vi "PicoScopeospaAdvancedTriggerPWQ.vi"(0 "handle in":i16=16384, 1 "Pulse Width Qualifier Settings":T3 {"Pulse Width Type" items=["None", "Less Than", "Greater Than", "In Range", "Out of Range"]}, 2 "Pulse Width Qualifier Trigger Properties":T1={"Channel A Trigger Properties"={"Threshold Mode"=0, "Available"=TRUE, "Direction"=2}, "Channel B Trigger Properties"={"Threshold Mode"=0, "Available"=FALSE, "Direction"=2}, "Channel C Trigger Properties"={"Threshold Mode"=0, "Available"=FALSE, "Direction"=2}, "Channel D Trigger Properties"={"Threshold Mode"=0, "Available"=FALSE, "Direction"=2}, "Channel E Trigger Properties"={"Threshold Mode"=0, "Available"=FALSE, "Direction"=2}, "Channel F Trigger Properties"={"Threshold Mode"=0, "Available"=FALSE, "Direction"=2}, "Channel G Trigger Properties"={"Threshold Mode"=0, "Available"=FALSE, "Direction"=2}, "Channel H Trigger Properties"={"Threshold Mode"=0, "Available"=FALSE, "Direction"=2}, "Port 0 Trigger Properties"={"Threshold Mode"=0, "Available"=FALSE, "Direction"=2}, "Port 1 Trigger Properties"={"Threshold Mode"=0, "Available"=FALSE, "Direction"=2}} {"Port 1 Trigger Properties"."Direction" items=["Rising"=2, "Falling"=3, "Rising Lower"=7, "Above"=0, "Below"=1, "Rising or Falling"=4, "Falling Lower"=8, "Below Lower"=6, "Above Lower"=5]; "Port 1 Trigger Properties"."Threshold Mode" items=["Level", "Window"]; "Port 0 Trigger Properties"."Direction" items=["Rising"=2, "Falling"=3, "Rising Lower"=7, "Above"=0, "Below"=1, "Rising or Falling"=4, "Falling Lower"=8, "Below Lower"=6, "Above Lower"=5]; "Port 0 Trigger Properties"."Threshold Mode" items=["Level", "Window"]; "Channel H Trigger Properties"."Direction" items=["Rising"=2, "Falling"=3, "Rising Lower"=7, "Above"=0, "Below"=1, "Rising or Falling"=4, "Falling Lower"=8, "Below Lower"=6, "Above Lower"=5]; "Channel H Trigger Properties"."Threshold Mode" items=["Level", "Window"]; "Channel G Trigger Properties"."Direction" items=["Rising"=2, "Falling"=3, "Rising Lower"=7, "Above"=0, "Below"=1, "Rising or Falling"=4, "Falling Lower"=8, "Below Lower"=6, "Above Lower"=5]; "Channel G Trigger Properties"."Threshold Mode" items=["Level", "Window"]; "Channel F Trigger Properties"."Direction" items=["Rising"=2, "Falling"=3, "Rising Lower"=7, "Above"=0, "Below"=1, "Rising or Falling"=4, "Falling Lower"=8, "Below Lower"=6, "Above Lower"=5]; "Channel F Trigger Properties"."Threshold Mode" items=["Level", "Window"]; "Channel E Trigger Properties"."Direction" items=["Rising"=2, "Falling"=3, "Rising Lower"=7, "Above"=0, "Below"=1, "Rising or Falling"=4, "Falling Lower"=8, "Below Lower"=6, "Above Lower"=5]; "Channel E Trigger Properties"."Threshold Mode" items=["Level", "Window"]; "Channel D Trigger Properties"."Direction" items=["Rising"=2, "Falling"=3, "Rising Lower"=7, "Above"=0, "Below"=1, "Rising or Falling"=4, "Falling Lower"=8, "Below Lower"=6, "Above Lower"=5]; "Channel D Trigger Properties"."Threshold Mode" items=["Level", "Window"]; "Channel C Trigger Properties"."Direction" items=["Rising"=2, "Falling"=3, "Rising Lower"=7, "Above"=0, "Below"=1, "Rising or Falling"=4, "Falling Lower"=8, "Below Lower"=6, "Above Lower"=5]; "Channel C Trigger Properties"."Threshold Mode" items=["Level", "Window"]; "Channel B Trigger Properties"."Direction" items=["Rising"=2, "Falling"=3, "Rising Lower"=7, "Above"=0, "Below"=1, "Rising or Falling"=4, "Falling Lower"=8, "Below Lower"=6, "Above Lower"=5]; "Channel B Trigger Properties"."Threshold Mode" items=["Level", "Window"]; "Channel A Trigger Properties"."Direction" items=["Rising"=2, "Falling"=3, "Rising Lower"=7, "Above"=0, "Below"=1, "Rising or Falling"=4, "Falling Lower"=8, "Below Lower"=6, "Above Lower"=5]; "Channel A Trigger Properties"."Threshold Mode" items=["Level", "Window"]}, 11 "error in":errorcluster, 13 "Pulse Width Qualifier Conditions":T2 {"Port 1" items=["Don't Care", "True", "False"]; "Channel H" items=["Don't Care", "True", "False"]; "Channel G" items=["Don't Care", "True", "False"]; "Channel F" items=["Don't Care", "True", "False"]; "Channel E" items=["Don't Care", "True", "False"]; "Aux" items=["Don't Care", "True", "False"]; "Port 0" items=["Don't Care", "True", "False"]; "Channel D" items=["Don't Care", "True", "False"]; "Channel C" items=["Don't Care", "True", "False"]; "Channel B" items=["Don't Care", "True", "False"]; "Channel A" items=["Don't Care", "True", "False"]; "Condition Logic" items=["AND", "OR", "XOR"]}) -> (4 "handle out":i16=16384, 15 "error out":errorcluster)   [LabVIEW 2010]
doc: "This sub VI is an interface for the advanced trigger features of the oscilloscope to support Pulse width qualifier (PWQ)."
uses:
  ps6000a.dll
  psospa.dll
panel:
  in  "PWQ Info Action XOR":bool=TRUE
  in  "PWQ Info Action OR":bool=TRUE
  # "For Condition Logic Suggested settings;\nFor AND, XOR logic-(parallel triggers)\nUse level-type triggers (Level or Inside/outside Window Triggers)\n\nFor OR logic- (single channel)\nUse edge types (e.g. rising, falling, entering window)"
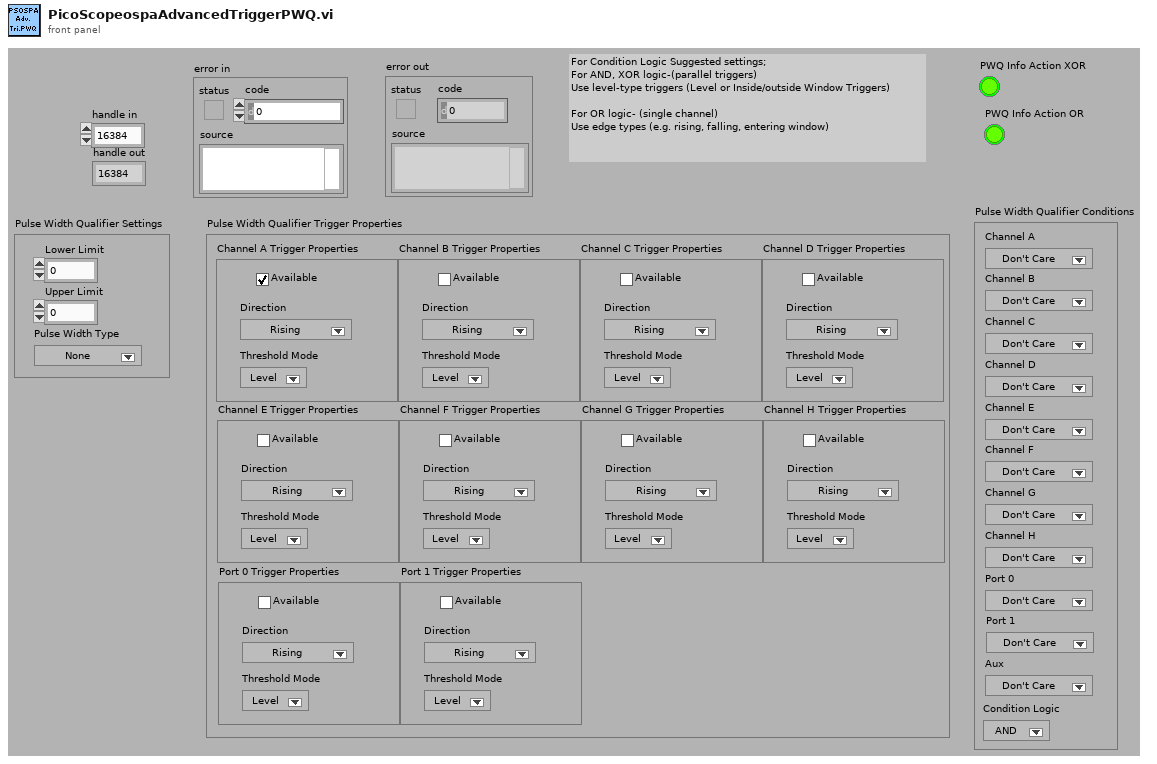
[diagram p1: front panel]
types:
  T1 = cluster{"Channel A Trigger Properties":cluster{"Threshold Mode":i32, "Available":bool, "Direction":u32}, "Channel B Trigger Properties":cluster{"Threshold Mode":i32, "Available":bool, "Direction":u32}, "Channel C Trigger Properties":cluster{"Threshold Mode":i32, "Available":bool, "Direction":u32}, "Channel D Trigger Properties":cluster{"Threshold Mode":i32, "Available":bool, "Direction":u32}, "Channel E Trigger Properties":cluster{"Threshold Mode":i32, "Available":bool, "Direction":u32}, "Channel F Trigger Properties":cluster{"Threshold Mode":i32, "Available":bool, "Direction":u32}, "Channel G Trigger Properties":cluster{"Threshold Mode":i32, "Available":bool, "Direction":u32}, "Channel H Trigger Properties":cluster{"Threshold Mode":i32, "Available":bool, "Direction":u32}, "Port 0 Trigger Properties":cluster{"Threshold Mode":i32, "Available":bool, "Direction":u32}, "Port 1 Trigger Properties":cluster{"Threshold Mode":i32, "Available":bool, "Direction":u32}}
  T2 = cluster{"Channel A":u16, "Channel B":u16, "Channel C":u16, "Channel D":u16, "Channel E":u16, "Channel F":u16, "Channel G":u16, "Channel H":u16, "Port 0":u16, "Port 1":u16, "Aux":u16, "Condition Logic":u16}
  T3 = cluster{"Lower Limit":u32, "Upper Limit":u32, "Pulse Width Type":u32}
  T4 = cluster{"status":bool, "code":u32, "source":string}
  T5 = cluster{"Threshold Mode":i32, "Available":bool, "Direction":u32}[]
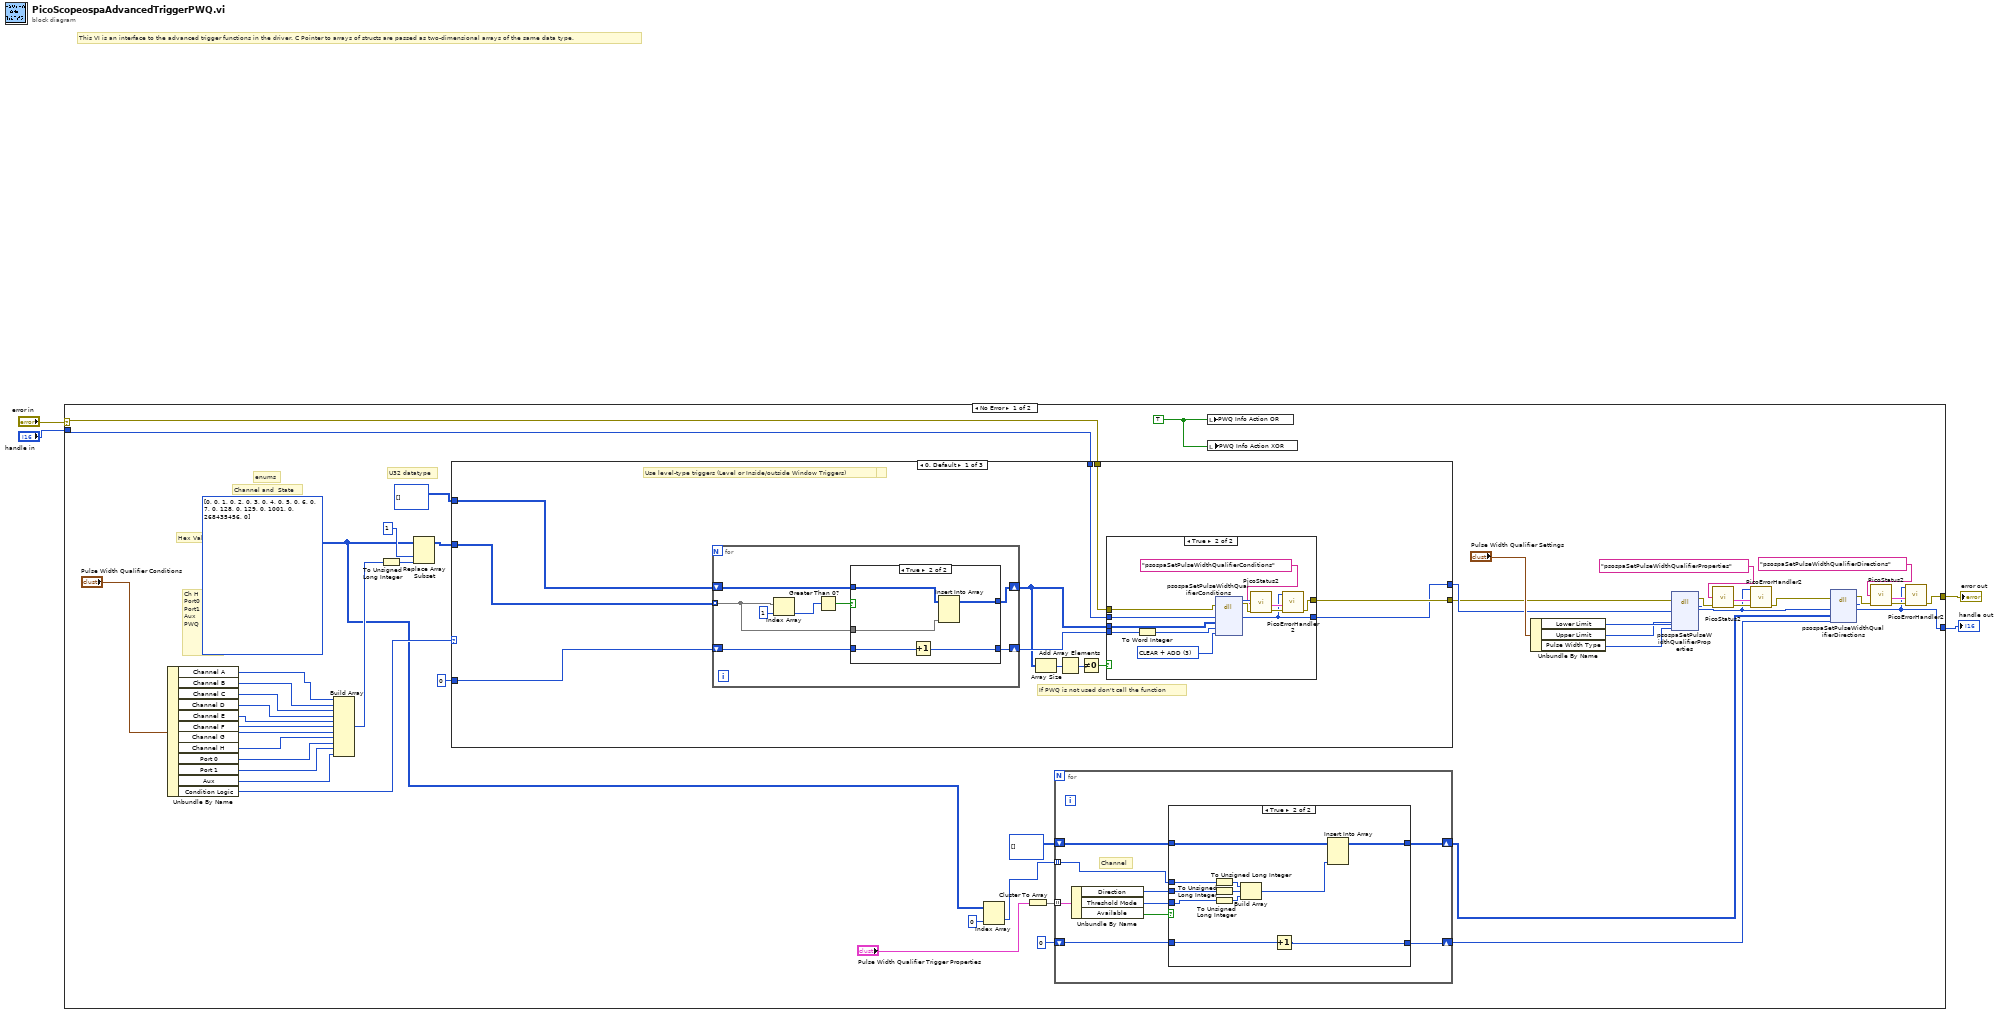
[diagram p0: block diagram]
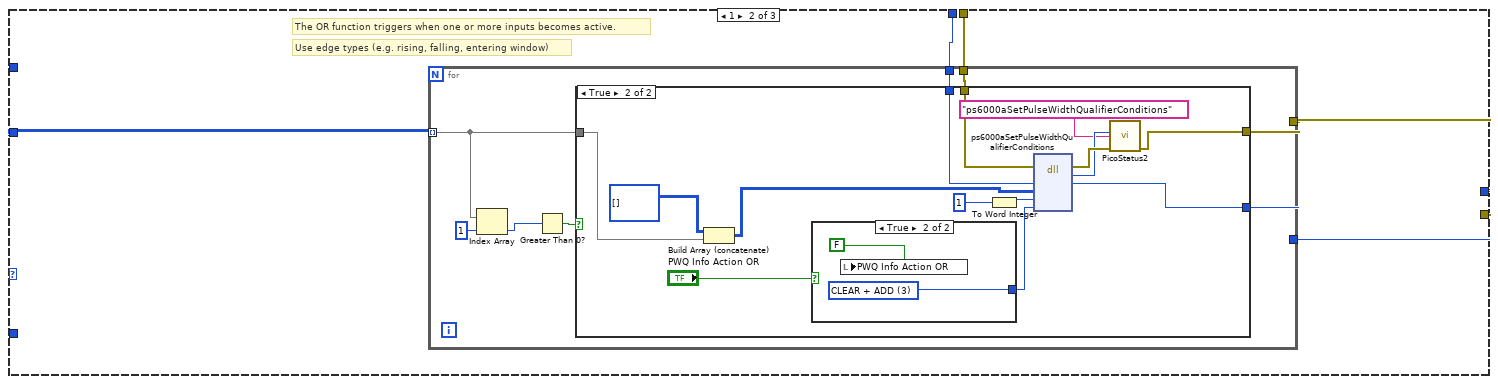
[diagram p5: hidden frame]
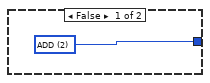
[diagram p7: hidden frame]
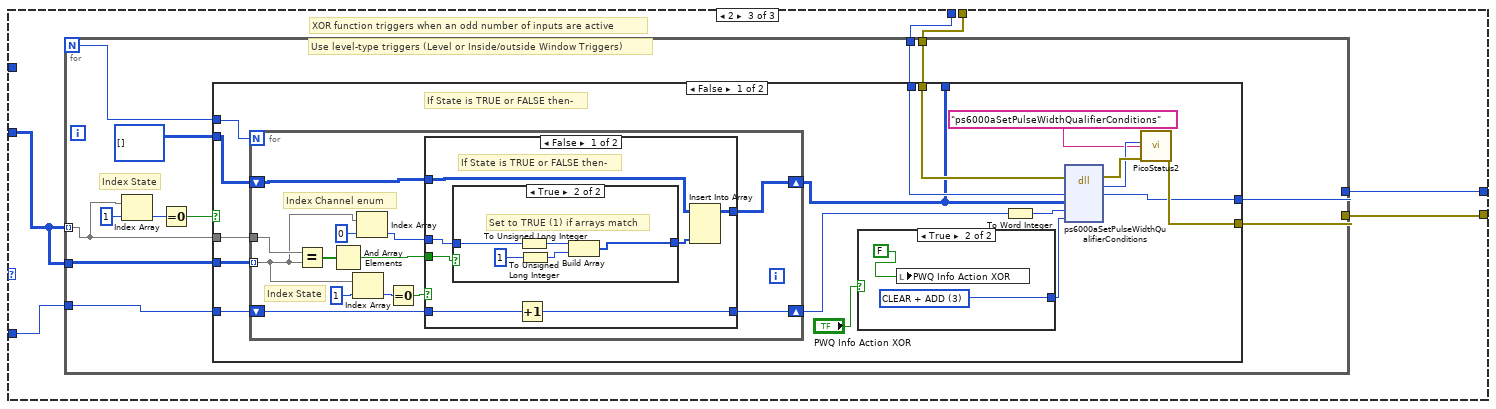
[diagram p8: hidden frame]
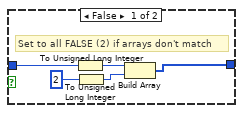
[diagram p9: hidden frame]
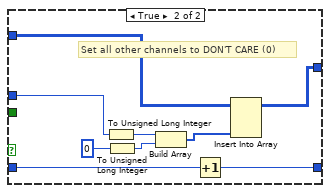
[diagram p10: hidden frame]
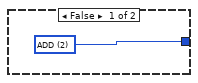
[diagram p11: hidden frame]
diagram:
  # "This VI is an interface to the advanced trigger functions in the driver. C Pointer to arrays of structs are passed as two-dimensional arrays of the same data type."
  n1 = case shown="No Error" "error in" {
    selector: "error in" -> [w14 w232]
    tunnel: "handle in" -> [w13 w233]
    tunnel: [w6 w233] -> w2
    tunnel: [w12 w232] -> w1
    frame No Error {
      w30 = TRUE ("PWQ Info Action XOR")
      w15 = u32[][] [[0, 0], [1, 0], [2, 0], [3, 0], [4, 0], [5, 0], [6, 0], [7, 0], [128, 0], [129, 0], [1001, 0], [268435456, 0]]
      # "U32 datatype"
      # "enums"
      # "Ch H\nPort0\nPort1\nAux\nPWQ"
      # "Channel and  State"
      # "Hex Values"
      n2 = Unbundle By Name("Pulse Width Qualifier Conditions") -> ("Channel A"=w40:u16, "Channel B"=w39:u16, "Channel C"=w38:u16, "Channel D"=w37:u16, "Channel E"=w36:u16, "Channel F"=w35:u16, "Channel G"=w34:u16, "Channel H"=w33:u16, "Port 0"=w32:u16, "Port 1"=w31:u16, "Aux"=w16:u16, "Condition Logic"=w17:u16)
      n3 = Build Array(w40, w39, w38, w37, w36, w35, w34, w33, w32, w31, w16) -> (w54:u16[])
      n4 = To Unsigned Long Integer(number=w54) -> (unsigned 32bit integer=w43:u32[])
      n5 = Replace Array Subset(array=w15, new element=w43, index (col)=1 ("disabled index (col)")) -> (w42:u32[][])  [unwired: 1 in]
      n6 = case shown="0, Default" w17 {
        tunnel: u32[][] [] -> [w89 _ _]
        tunnel: i16 0 -> [w88 _ w152]
        tunnel: w14 -> [w85 w124 w157]
        tunnel: w13 -> [w84 w123 w156]
        tunnel: [w83 w122 w155] -> w44
        tunnel: [w82 w121 w154] -> w45
        tunnel: w42 -> [w86 w120 w153]
        frame 0, Default {
          # "If PWQ is not used don't call the function"
          # "AND function requires both inputs to be active before it will trigger."
          # "Use level-type triggers (Level or Inside/outside Window Triggers)"
          n7 = for {
            shift-right: [w111] -> w87
            shift-left: w88 -> [w110]
            shift-right: [w109] -> w81
            shift-left: w89 -> [w112]
            tunnel: w86 -> [w107] mode=indexing
            n8 = Index Array(array=w107, index=1) -> (element=w106:u32)
            n9 = Greater Than 0?(x=w106) -> (x > 0?=w108:bool)
            n10 = case shown="True" w108 {
              tunnel: w112 -> [w114 w119]
              tunnel: [w114 w118] -> w109
              tunnel: [w113 w117] -> w111
              tunnel: w110 -> [w113 w116]
              tunnel: w107 -> [_ w115]
              frame False {
              }
              frame True {
                n11 = Increment(x=w116) -> (x+1=w117:i16)
                n12 = Insert Into Array(array=w119, new element=w115) -> (w118:u32[][])  [unwired: 2 in]
              }
            }
          }
          n13 = Array Size(array=w81) -> (size(s)=w79:i32[])
          n14 = Add Array Elements(numeric array=w79) -> (sum=w80:i32)
          n15 = Not Equal To 0?(x=w80) -> (x != 0?=w78:bool)
          n16 = case shown="True" w78 {
            tunnel: w87 -> [_ w104]
            tunnel: w85 -> [w91 w100]
            tunnel: w84 -> [w90 w99]
            tunnel: w81 -> [_ w96]
            tunnel: [w91 w95] -> w83
            tunnel: [w90 w92] -> w82
            frame False {
            }
            frame True {
              w98 = u32 3 items=["CLEAR + ADD"=3, "CLEAR"=1, "ADD"=2] ("Condition Action")
              n17 = To Word Integer(number=w104) -> (16bit integer=w97:i16)
              n18 = dll-call lib="psospa.dll" fn="psospaSetPulseWidthQualifierConditions" ("ps3000.dll:_ps3000_open_unit@0")(error in=w100, "handle"=w99, "conditions"=w96, "nConditions"=w97, "action"=w98) -> (error out=w103:errorcluster, "PICO_STATUS"=w102:u32, "handle"=w92:i16)  [unwired: 5 in, 1 out]
              n19 = call "PicoStatus2.vi"("PICO source"="psospaSetPulseWidthQualifierConditions" ("source"), "Error in"=w103, "PICO STATUS"=w102) -> ("error out"=w94:errorcluster, "PICO_STATUS out"=w93:T4)  [unwired: 5 in]
              n20 = call "PicoErrorHandler2.vi"("error in (no error)"=w94, "PICO_STATUS in"=w93, "handle In"=w92) -> ("error out"=w95:errorcluster)  [unwired: 8 in]
            }
          }
        }
        frame 1 {
          # "Use edge types (e.g. rising, falling, entering window)"
          # "The OR function triggers when one or more inputs becomes active."
          n21 = for {
            tunnel: w124 -> [w132]
            tunnel: w123 -> [w131]
            tunnel: [w130] -> w122
            tunnel: [w129] -> w121
            tunnel: w120 -> [w127] mode=indexing
            n22 = Index Array(array=w127, index=1) -> (element=w126:u32)
            n23 = Greater Than 0?(x=w126) -> (x > 0?=w125:bool)
            n24 = case shown="True" w125 {
              tunnel: w132 -> [w133 w144]
              tunnel: w131 -> [w134 w143]
              tunnel: [w133 w141] -> w130
              tunnel: [w134 w140] -> w129
              tunnel: w127 -> [_ w135]
              frame False {
              }
              frame True {
                n25 = Build Array (concatenate)(u32[][] [], w135) -> (w137:u32[][])
                n26 = case shown="True" "PWQ Info Action OR" {
                  tunnel: [w149 w151] -> w142
                  frame False {
                    w149 = u32 2 items=["CLEAR"=1, "ADD"=2, "CLEAR + ADD"=3] ("Condition Action")
                  }
                  frame True {
                    w151 = u32 3 items=["CLEAR"=1, "ADD"=2, "CLEAR + ADD"=3] ("Condition Action")
                    n27 = local write "PWQ Info Action OR"(FALSE ("Boolean")) -> ()
                  }
                }
                n28 = To Word Integer(number=i16 1) -> (16bit integer=w148:i16)
                n29 = dll-call lib="ps6000a.dll" fn="ps6000aSetPulseWidthQualifierConditions" ("ps3000.dll:_ps3000_open_unit@0")(error in=w144, "handle"=w143, "conditions"=w137, "nConditions"=w148, "action"=w142) -> (error out=w147:errorcluster, "PICO_STATUS"=w146:u32, "handle"=w140:i16)  [unwired: 5 in, 1 out]
                n30 = call "PicoStatus2.vi"("PICO source"="ps6000aSetPulseWidthQualifierConditions" ("source"), "Error in"=w147, "PICO STATUS"=w146) -> ("error out"=w141:errorcluster)  [unwired: 5 in, 1 out]
              }
            }
          }
        }
        frame 2 {
          # "Use level-type triggers (Level or Inside/outside Window Triggers)"
          # "XOR function triggers when an odd number of inputs are active"
          n31 = for {
            N -> [w165]
            tunnel: w157 -> [w169]
            tunnel: w156 -> [w168]
            tunnel: [w167] -> w155
            tunnel: [w166] -> w154
            tunnel: w153 -> [w159] mode=indexing
            tunnel: w153 -> [w162]
            tunnel: w152 -> [w163]
            # "Index State"
            n32 = Index Array(array=w159, index=1) -> (element=w160:u32)
            n33 = Equal To 0?(x=w160) -> (x = 0?=w158:bool)
            n34 = case shown="False" w158 {
              tunnel: w169 -> [w186 w229]
              tunnel: w168 -> [w185 w230]
              tunnel: [w184 w229] -> w167
              tunnel: [w183 w230] -> w166
              tunnel: [w181 w231] -> _
              tunnel: w165 -> [w180 _]
              tunnel: u32[][] [] -> [w179 w231]
              tunnel: w163 -> [w178 _]
              tunnel: w162 -> [w177 _]
              tunnel: w159 -> [w176 _]
              frame False {
                # "If State is TRUE or FALSE then-"
                n35 = for {
                  N: w180 -> [_]
                  shift-right: [w198] -> w182
                  shift-left: w178 -> [w199]
                  shift-right: [w187] -> w181
                  shift-left: w179 -> [w188]
                  tunnel: w176 -> [w195]
                  tunnel: w177 -> [w191] mode=indexing
                  # "Index State"
                  # "Index Channel enum"
                  n36 = Equal?(x=w195, y=w191) -> (x = y?=w189:bool[])
                  n37 = And Array Elements(Boolean array=w189) -> (logical AND=w194:bool)
                  n38 = Index Array(array=w191, index=1) -> (element=w192:u32)
                  n39 = Index Array(array=w191, index=0) -> (element=w196:u32)
                  n40 = Equal To 0?(x=w192) -> (x = 0?=w190:bool)
                  n41 = case shown="False" w190 {
                    tunnel: w199 -> [w206 w217]
                    tunnel: [w205 w218] -> w198
                    tunnel: w196 -> [w204 w221]
                    tunnel: w194 -> [w203 _]
                    tunnel: w188 -> [w202 w220]
                    tunnel: [w200 w219] -> w187
                    frame False {
                      # "If State is TRUE or FALSE then-"
                      n42 = case shown="True" w203 {
                        tunnel: [w211 w216] -> w201
                        tunnel: w204 -> [w210 w215]
                        frame False {
                          # "Set to all FALSE (2) if arrays don't match"
                          n43 = To Unsigned Long Integer(number=w210) -> (unsigned 32bit integer=w208:u32)
                          n44 = To Unsigned Long Integer(number=u32 2) -> (unsigned 32bit integer=w209:u32)
                          n45 = Build Array(w208, w209) -> (w211:u32[])
                        }
                        frame True {
                          # "Set to TRUE (1) if arrays match"
                          n46 = To Unsigned Long Integer(number=w215) -> (unsigned 32bit integer=w213:u32)
                          n47 = To Unsigned Long Integer(number=u32 1) -> (unsigned 32bit integer=w214:u32)
                          n48 = Build Array(w213, w214) -> (w216:u32[])
                        }
                      }
                      n49 = Increment(x=w206) -> (x+1=w205:i16)
                      n50 = Insert Into Array(array=w202, new element=w201) -> (w200:u32[][])  [unwired: 2 in]
                    }
                    frame True {
                      # "Set all other channels to DON'T CARE (0)"
                      n51 = To Unsigned Long Integer(number=w221) -> (unsigned 32bit integer=w223:u32)
                      n52 = To Unsigned Long Integer(number=u32 0) -> (unsigned 32bit integer=w224:u32)
                      n53 = Build Array(w223, w224) -> (w225:u32[])
                      n54 = Increment(x=w217) -> (x+1=w218:i16)
                      n55 = Insert Into Array(array=w220, new element=w225) -> (w219:u32[][])  [unwired: 2 in]
                    }
                  }
                }
                n56 = case shown="True" "PWQ Info Action XOR" {
                  tunnel: [w226 w228] -> w170
                  frame False {
                    w226 = u32 2 items=["CLEAR + ADD"=3, "CLEAR"=1, "ADD"=2] ("Condition Action")
                  }
                  frame True {
                    w228 = u32 3 items=["CLEAR + ADD"=3, "CLEAR"=1, "ADD"=2] ("Condition Action")
                    n57 = local write "PWQ Info Action XOR"(FALSE ("Boolean")) -> ()
                  }
                }
                n58 = To Word Integer(number=w182) -> (16bit integer=w175:i16)
                n59 = dll-call lib="ps6000a.dll" fn="ps6000aSetPulseWidthQualifierConditions" ("ps3000.dll:_ps3000_open_unit@0")(error in=w186, "handle"=w185, "conditions"=w181, "nConditions"=w175, "action"=w170) -> (error out=w174:errorcluster, "PICO_STATUS"=w173:u32, "handle"=w183:i16)  [unwired: 5 in, 1 out]
                n60 = call "PicoStatus2.vi"("PICO source"="ps6000aSetPulseWidthQualifierConditions" ("source"), "Error in"=w174, "PICO STATUS"=w173) -> ("error out"=w184:errorcluster)  [unwired: 5 in, 1 out]
              }
              frame True {
              }
            }
          }
        }
      }
      n61 = Index Array(array=w15, index (col)=0 ("disabled index (col)")) -> (element=w18:u32[])  [unwired: 1 in]
      n62 = Cluster To Array(cluster="Pulse Width Qualifier Trigger Properties") -> (array=w24:T5)
      n63 = for {
        tunnel: w24 -> [w64] mode=indexing
        shift-right: [w59] -> w22
        shift-left: u32[][] [] -> [w60]
        shift-right: [w57] -> w20
        shift-left: i16 0 ("nDirections") -> [w58]
        tunnel: w18 -> [w56] mode=indexing
        # "Channel"
        n64 = Unbundle By Name(w64) -> ("Direction"=w62:u32, "Threshold Mode"=w61:i32, "Available"=w63:bool)
        n65 = case shown="True" w63 {
          tunnel: w56 -> [_ w73]
          tunnel: w62 -> [_ w72]
          tunnel: w61 -> [_ w71]
          tunnel: w60 -> [w66 w70]
          tunnel: [w66 w69] -> w59
          tunnel: [w65 w68] -> w57
          tunnel: w58 -> [w65 w67]
          frame False {
          }
          frame True {
            n66 = To Unsigned Long Integer(number=w73) -> (unsigned 32bit integer=w75:u32)
            n67 = To Unsigned Long Integer(number=w72) -> (unsigned 32bit integer=w76:u32)
            n68 = To Unsigned Long Integer(number=w71) -> (unsigned 32bit integer=w74:u32)
            n69 = Build Array(w75, w76, w74) -> (w77:u32[])
            n70 = Increment(x=w67) -> (x+1=w68:i16)
            n71 = Insert Into Array(array=w70, new element=w77) -> (w69:u32[][])  [unwired: 2 in]
          }
        }
      }
      n72 = local write "PWQ Info Action OR"(w30) -> ()
      n73 = local write "PWQ Info Action XOR"(w30) -> ()
      n74 = Unbundle By Name("Pulse Width Qualifier Settings") -> ("Lower Limit"=w51:u32, "Upper Limit"=w50:u32, "Pulse Width Type"=w49:u32)
      n75 = dll-call lib="psospa.dll" fn="psospaSetPulseWidthQualifierProperties" ("ps3000.dll:_ps3000_open_unit@0")(error in=w44, "handle"=w45, "lower"=w51, "upper"=w50, "type"=w49) -> (error out=w53:errorcluster, "PICO_STATUS"=w48:u32, "handle"=w5:i16)  [unwired: 5 in, 1 out]
      n76 = call "PicoStatus2.vi"("PICO source"="psospaSetPulseWidthQualifierProperties" ("source"), "Error in"=w53, "PICO STATUS"=w48) -> ("error out"=w9:errorcluster, "PICO_STATUS out"=w8:T4)  [unwired: 5 in]
      n77 = call "PicoErrorHandler2.vi"("error in (no error)"=w9, "PICO_STATUS in"=w8, "handle In"=w5) -> ("error out"=w7:errorcluster)  [unwired: 8 in]
      n78 = dll-call lib="psospa.dll" fn="psospaSetPulseWidthQualifierDirections" ("ps3000.dll:_ps3000_open_unit@0")(error in=w7, "handle"=w5, "directions"=w22, "nDirections"=w20) -> (error out=w29:errorcluster, "PICO_STATUS"=w28:u32, "handle"=w6:i16)  [unwired: 4 in, 1 out]
      n79 = call "PicoStatus2.vi"("PICO source"="psospaSetPulseWidthQualifierDirections" ("source"), "Error in"=w29, "PICO STATUS"=w28) -> ("error out"=w11:errorcluster, "PICO_STATUS out"=w10:T4)  [unwired: 5 in]
      n80 = call "PicoErrorHandler2.vi"("error in (no error)"=w11, "PICO_STATUS in"=w10, "handle In"=w6) -> ("error out"=w12:errorcluster)  [unwired: 8 in]
    }
    frame Error {
    }
  }
  "handle out" <- w2
  "error out" <- w1
